vi "Ohaus STX2201 (com1).vi"(4 "State":i16, 5 "Time":dbl format="%.2f", 6 "Sensor Values":dbl[](array[numeric]), 7 "Set Points":dbl[](array[numeric])) -> (0 "required data":T1, 3 "output value":dbl)   [LabVIEW 2019]
uses:
  <vilib>/Instr/_visa.llb/VISA Configure Serial Port (Instr).vi
panel:
  out "String":string
  out "VISA resource name out":refnum<visa-resource-name>
  # "Enter the correct information for this control code in the required data structure below. Then make the current value default by right clicking on the border of the data structure. Select \"data operations\" and then select \"make current value default\". These values will be displayed by process controller."
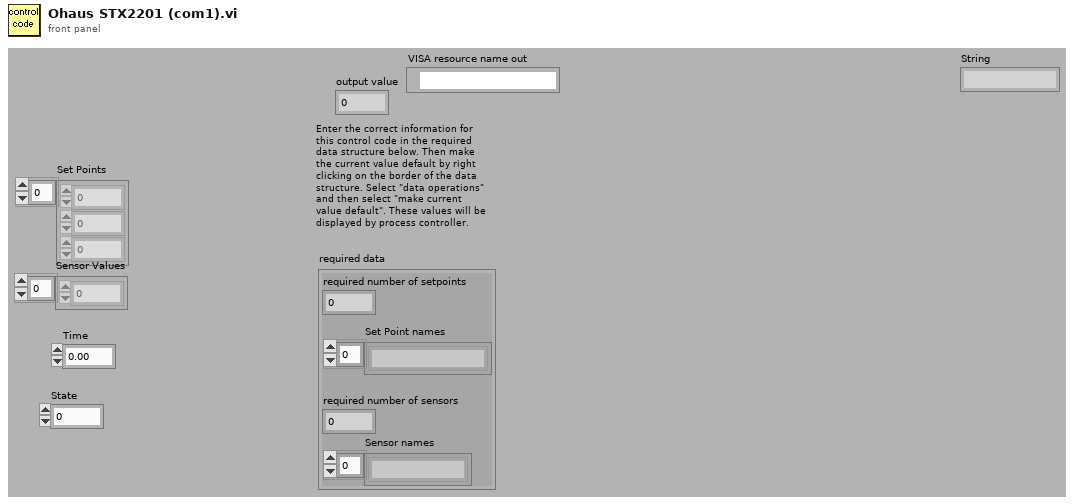
[diagram p1: front panel]
types:
  T1 = cluster{"Set Point names":string[], "required number of setpoints":u8, "required number of sensors":u8, "Sensor names":string[]}
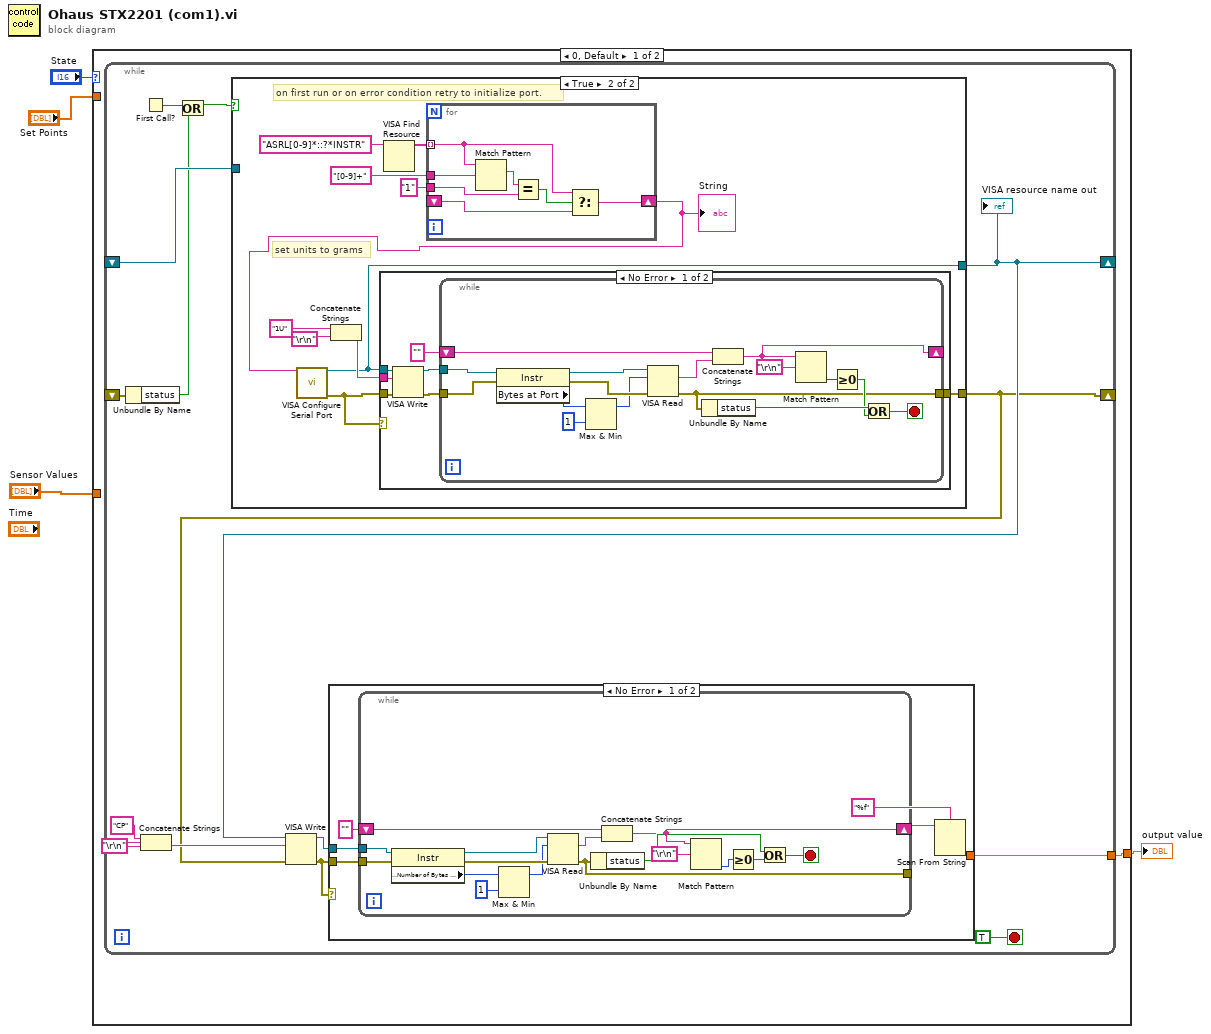
[diagram p0: block diagram]
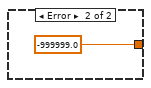
[diagram p2: hidden frame]
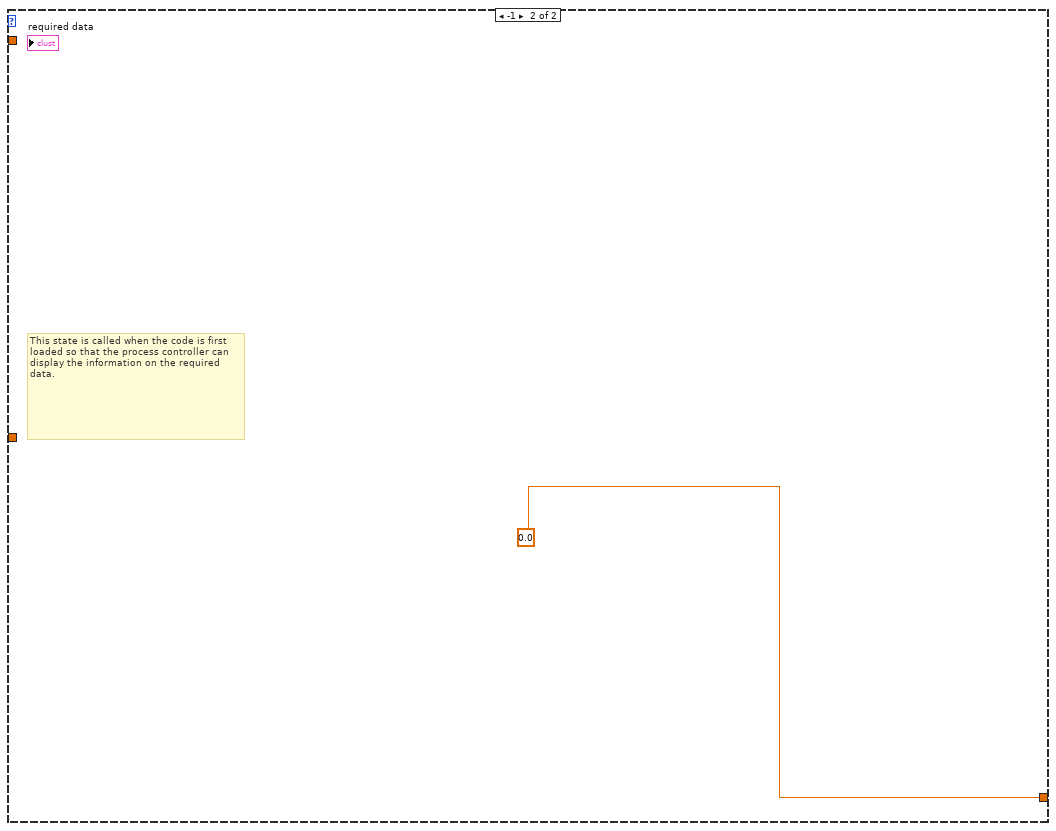
[diagram p5: hidden frame]
diagram:
  n1 = case shown="0, Default" "State" {
    tunnel: [w5 0.0 ("fraction on")] -> w3
    tunnel: "Set Points" -> [_ _]
    tunnel: "Sensor Values" -> [_ _]
    frame 0, Default {
      n2 = while {
        tunnel: [w19] -> w5
        shift-right: [w12] -> _
        shift-left: _ -> [w13]
        shift-right: [w10] -> _
        shift-left: _ -> [w9]
        stop <- TRUE stop-if-true
        n3 = Unbundle By Name(w9) -> ("status"=w7:bool)
        n4 = First Call?() -> (First Call?: T/F=w17:bool)
        n5 = Concatenate Strings("CP", "\r\n") -> (w14:string)
        n6 = Or(x=w17, y=w7) -> (x .or. y?=w8:bool)
        n7 = case shown="True" w8 {
          tunnel: [_ w51] -> w10
          tunnel: [w43 w46] -> w12
          tunnel: w13 -> [w43 _]
          frame False {
          }
          frame True {
            # "on first run or on error condition retry to initialize port."
            # "set units to grams"
            n8 = Concatenate Strings("1U", "\r\n") -> (w52:string)
            n9 = VISA Find Resource(11:"ASRL[0-9]*::?*INSTR" ("expression (\"?*\")")) -> (3:w49:string[])  [unwired: 2 in, 2 out]
            n10 = for {
              tunnel: w49 -> [w80] mode=indexing
              tunnel: "1" -> [w84]
              shift-right: [w81] -> w47
              shift-left: _ -> [w82]
              tunnel: "[0-9]+" ("regular expression") -> [w79]
              n11 = Match Pattern(string=w80, regular expression=w79) -> (match substring=w85:string)  [unwired: 1 in, 3 out]
              n12 = Equal?(x=w85, y=w84) -> (x = y?=w83:bool)
              n13 = Select(t=w80, s=w83, f=w82) -> (s? t:f=w81:string)
            }
            "String" <- w47
            n14 = call-poly "VISA Configure Serial Port"("VISA resource name"=w47) -> ("VISA resource name out"=w46:refnum<visa-resource-name>, "error out"=w45:errorcluster)  [unwired: 13 in]
            n15 = case shown="No Error" w45 {
              tunnel: w52 -> [w59 _]
              tunnel: w45 -> [w58 w78]
              tunnel: [w56 w78] -> w51
              tunnel: w46 -> [w55 _]
              frame No Error {
                n16 = VISA Write(VISA resource name=w55, write buffer=w59, error in (no error)=w58) -> (VISA resource name out=w57:refnum<visa-resource-name>, error out=w61:errorcluster)  [unwired: 1 out]
                n17 = while {
                  tunnel: w57 -> [w76]
                  tunnel: w61 -> [w74]
                  shift-right: [w63] -> _
                  shift-left: "" ("write buffer") -> [w77]
                  tunnel: [w62] -> w56
                  stop <- w72 stop-if-true
                  n18 = property class="Instr"(reference=w76, error in=w74) -> (reference out=w75:refnum<visa-resource-name>, error out=w73:errorcluster, "Bytes at Port"=w65:u32)
                  n19 = Max & Min(x=w65, y=u32 1) -> (max(x,y)=w66:u32)  [unwired: 1 out]
                  n20 = VISA Read(VISA resource name=w75, byte count=w66, error in (no error)=w73) -> (read buffer=w70:string, error out=w62:errorcluster)  [unwired: 2 out]
                  n21 = Unbundle By Name(w62) -> ("status"=w71:bool)
                  n22 = Concatenate Strings(w77, w70) -> (w63:string)
                  n23 = Match Pattern(string=w63, regular expression="\r\n") -> (offset past match=w68:i32)  [unwired: 1 in, 3 out]
                  n24 = Greater Or Equal To 0?(x=w68) -> (x >= 0?=w67:bool)
                  n25 = Or(x=w71, y=w67) -> (x .or. y?=w72:bool)
                }
              }
              frame Error {
              }
            }
          }
        }
        "VISA resource name out" <- w12
        n26 = VISA Write(VISA resource name=w12, write buffer=w14, error in (no error)=w10) -> (VISA resource name out=w18:refnum<visa-resource-name>, error out=w6:errorcluster)  [unwired: 1 out]
        n27 = case shown="No Error" w6 {
          tunnel: [w25 -999999.0] -> w19
          tunnel: w18 -> [w24 _]
          tunnel: w6 -> [w23 _]
          frame No Error {
            n28 = while {
              tunnel: w24 -> [w40]
              tunnel: w23 -> [w38]
              shift-right: [w26] -> w20
              shift-left: "" ("write buffer") -> [w41]
              tunnel: [w27] -> _
              stop <- w36 stop-if-true
              n29 = property class="Instr"(reference=w40, error in=w38) -> (reference out=w39:refnum<visa-resource-name>, error out=w37:errorcluster, "Serial Settings:Number of Bytes at Serial Port"=w29:u32)
              n30 = Max & Min(x=w29, y=u32 1) -> (max(x,y)=w30:u32)  [unwired: 1 out]
              n31 = VISA Read(VISA resource name=w39, byte count=w30, error in (no error)=w37) -> (read buffer=w34:string, error out=w27:errorcluster)  [unwired: 2 out]
              n32 = Unbundle By Name(w27) -> ("status"=w35:bool)
              n33 = Concatenate Strings(w41, w34) -> (w26:string)
              n34 = Match Pattern(string=w26, regular expression="\r\n") -> (offset past match=w32:i32)  [unwired: 1 in, 3 out]
              n35 = Greater Or Equal To 0?(x=w32) -> (x >= 0?=w31:bool)
              n36 = Or(x=w35, y=w31) -> (x .or. y?=w36:bool)
            }
            n37 = Scan From String(format string="%f", input string=w20) -> (output 1=w25:dbl)  [unwired: 3 in, 3 out]
          }
          frame Error {
          }
        }
      }
    }
    frame -1 {
      # "This state is called when the code is first loaded so that the process controller can display the information on the required data."
    }
  }
  "output value" <- w3
